vi "Set Properties from Initial.vi"(8 "error in(no error)":errorcluster, 10 "Initial Value":variant, 11 "Properties in":variant) -> (0 "error out":errorcluster, 2 "type":T1, 3 "Properties out":variant)   [LabVIEW 2020, in "Tag Engine Core.lvlib" / "Tag.lvclass"]
doc: "_SubVI_"
uses:
  Tag.lvclass
  <vilib>/Utility/Data Type/Type Definitions/Data Type.ctl
  Tag.lvclass/Tag.ctl
  <vilib>/Utility/Data Type/NI_Data Type.lvlib
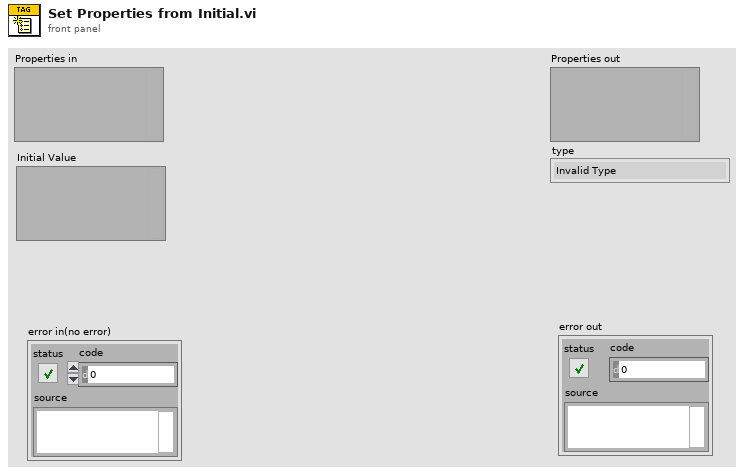
[diagram p1: front panel]
types:
  T1 = typedef "NI_Data Type.lvlib/Data Type.ctl" = enum8{"Invalid Type", "Void", "I8", "I16", "I32", "I64", "U8", "U16", "U32", "U64", "Single Float", "Double Float", "Extended Float", "Single Complex", "Double Complex", "Extended Complex", "Enum U8", "Enum U16", "Enum U32", "Enum U64", "Single Float With Unit", "Double Float With Unit", "Extended Float With Unit", "Single Complex with Unit", "Double Complex with Unit", "Extended Complex with Unit", "Boolean", "String", "Path", "Picture", "Tag", "Array", "Cluster", "Variant", "LV Variant", "Waveform", "Timestamp", "Digital Waveform", "Digital Data", "ExpressData", "Refnum", "External Data", "VI", "Poly VI", "LabVIEW Class Instance", "Fixed Point", "Set Collection", "Map Collection"}
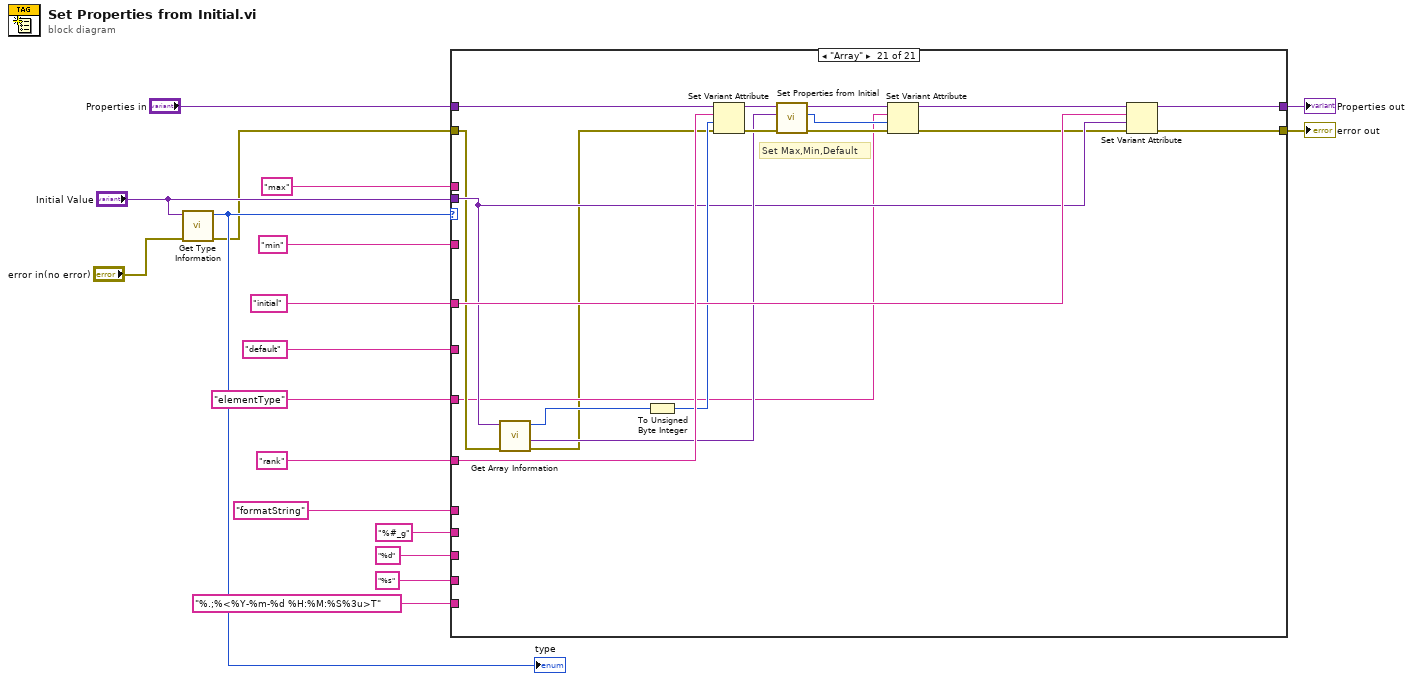
[diagram p0: block diagram]
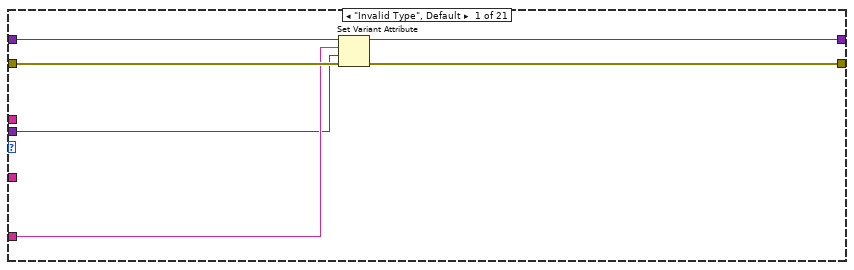
[diagram p2: hidden frame]
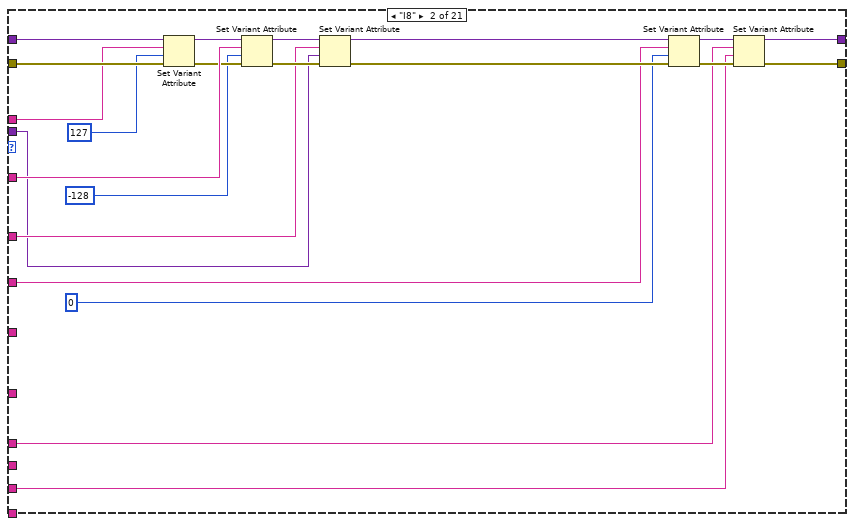
[diagram p3: hidden frame]
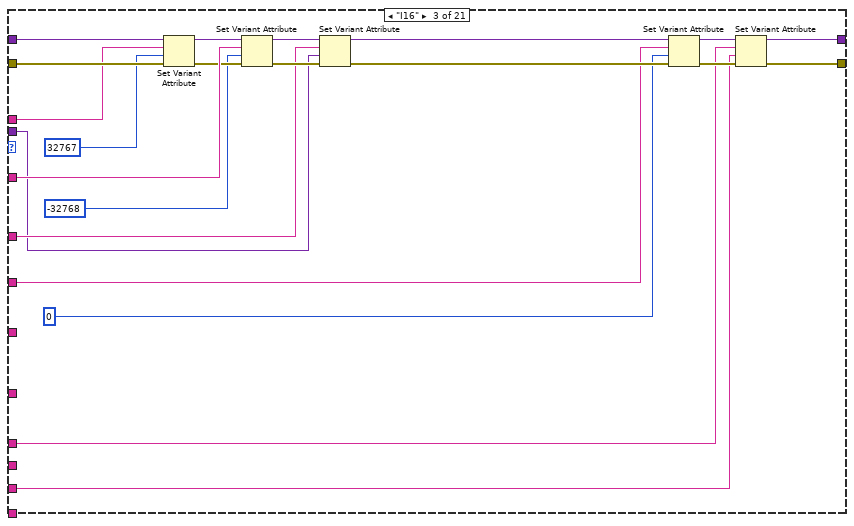
[diagram p4: hidden frame]
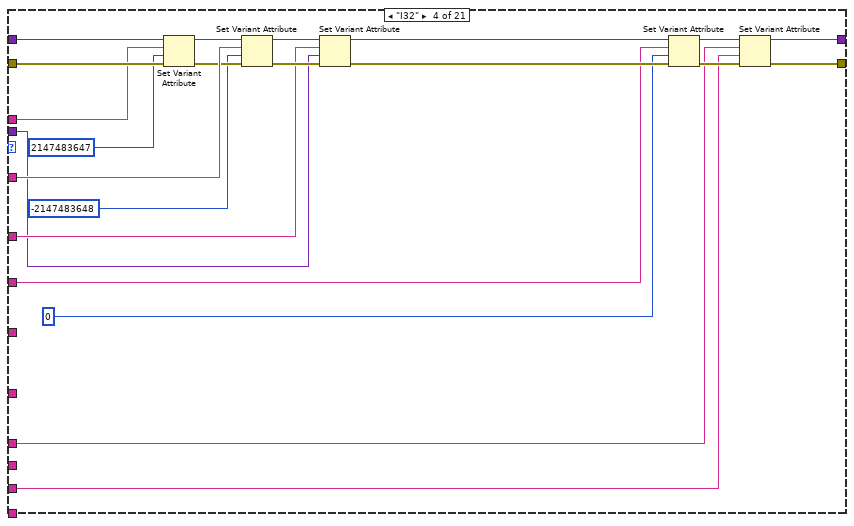
[diagram p5: hidden frame]
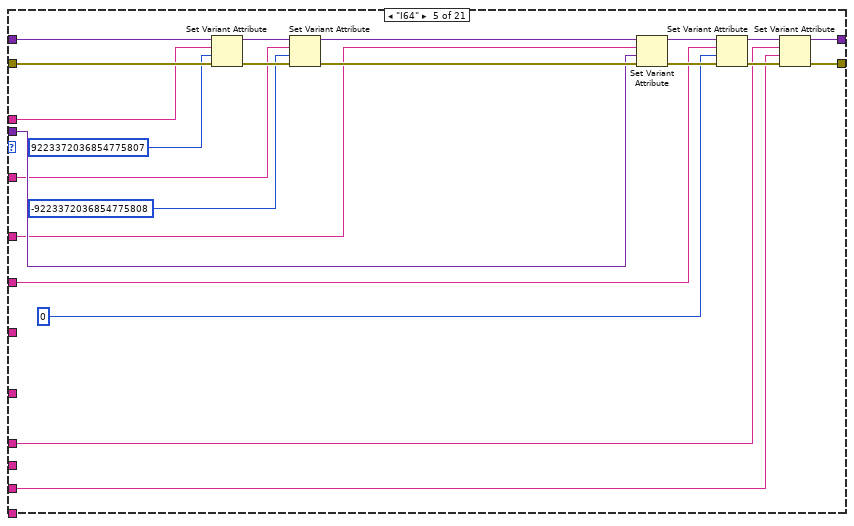
[diagram p6: hidden frame]
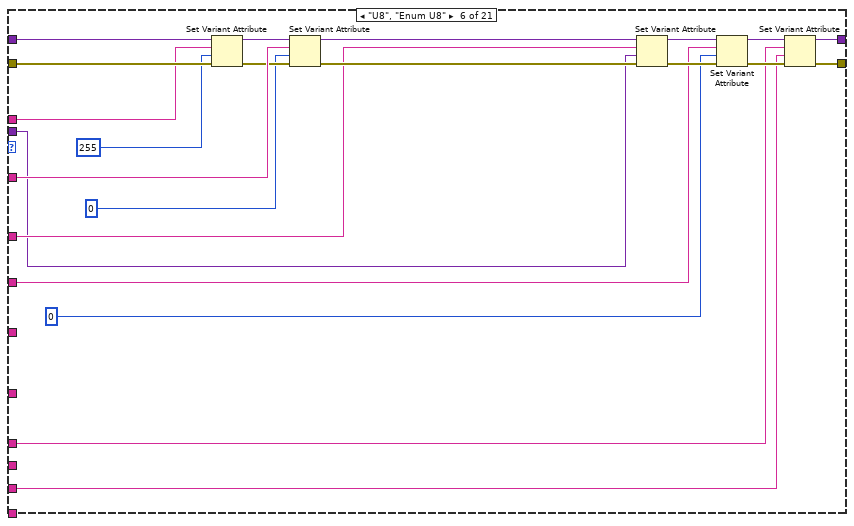
[diagram p7: hidden frame]
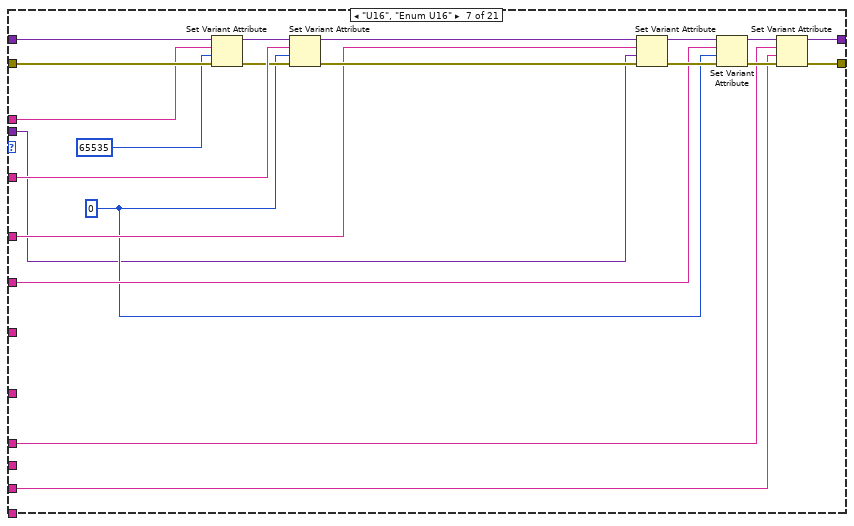
[diagram p8: hidden frame]
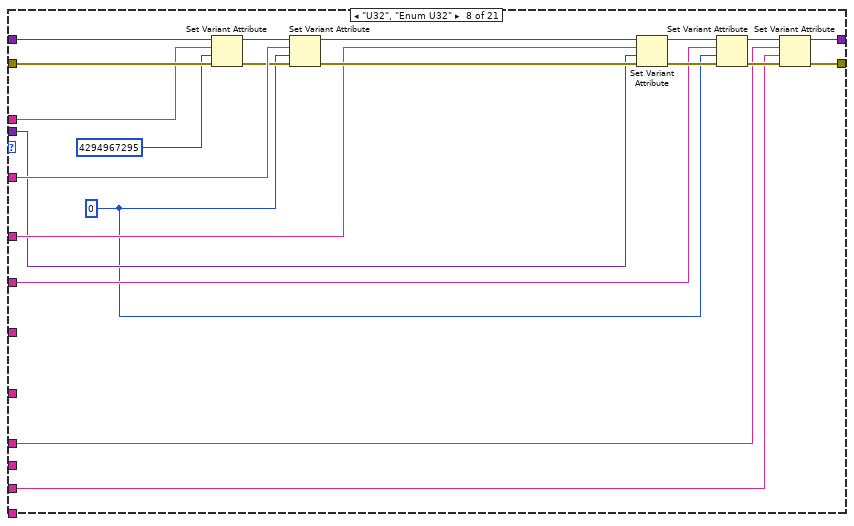
[diagram p9: hidden frame]
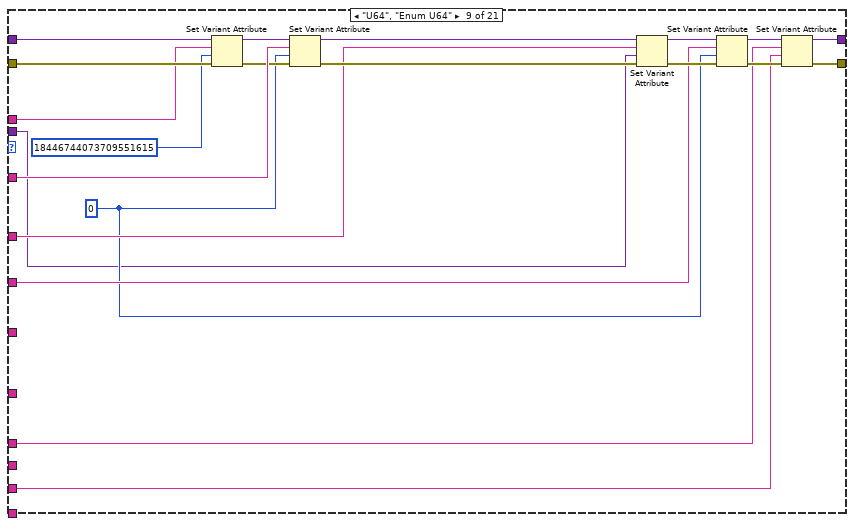
[diagram p10: hidden frame]
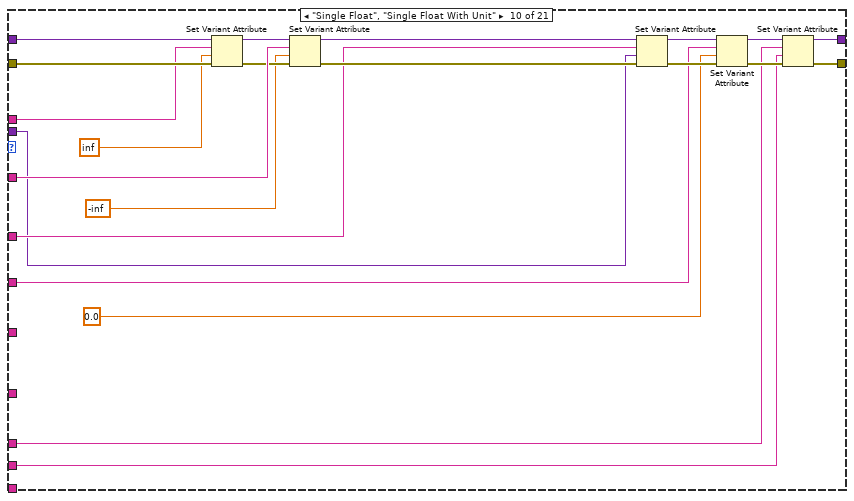
[diagram p11: hidden frame]
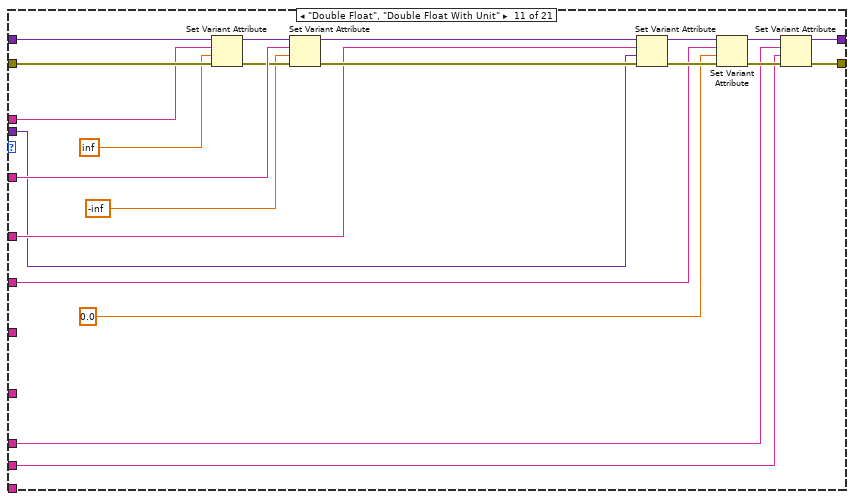
[diagram p12: hidden frame]
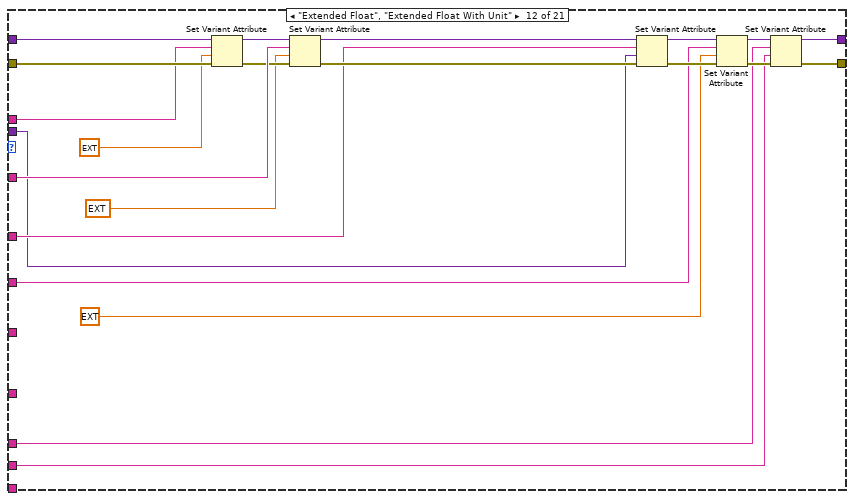
[diagram p13: hidden frame]
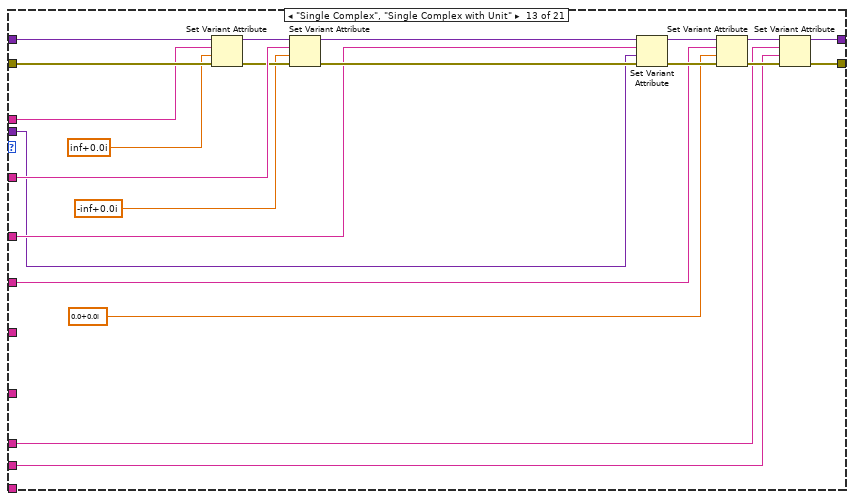
[diagram p14: hidden frame]
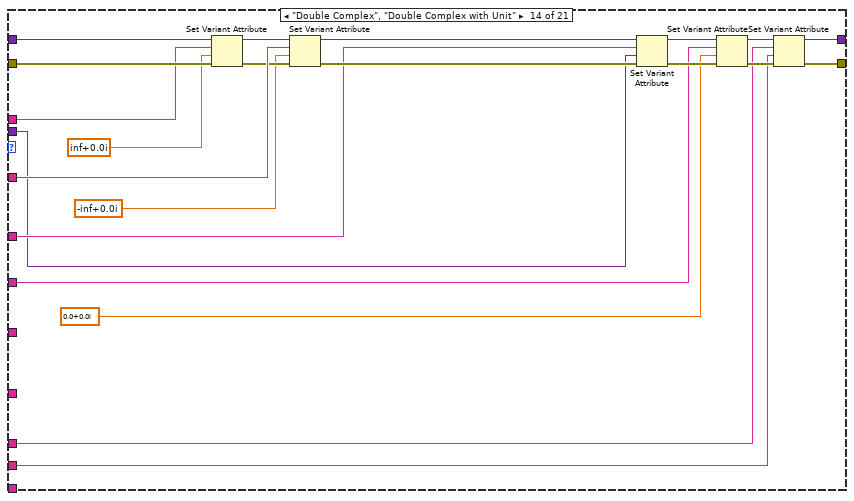
[diagram p15: hidden frame]
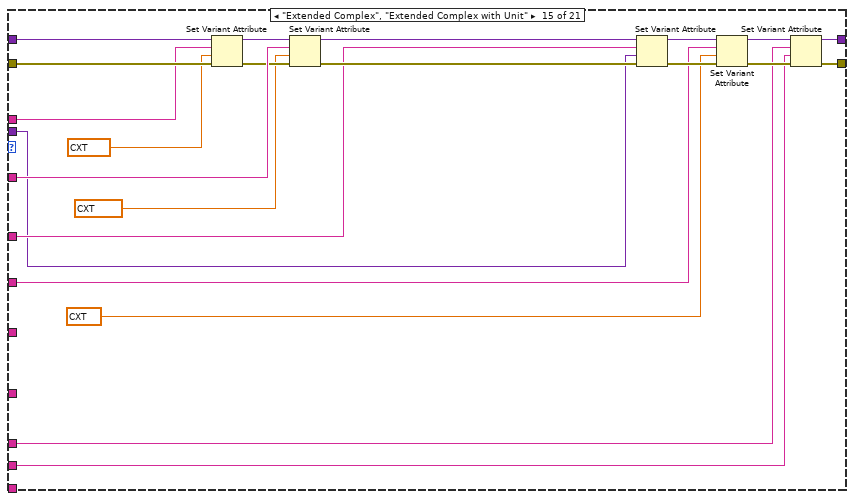
[diagram p16: hidden frame]
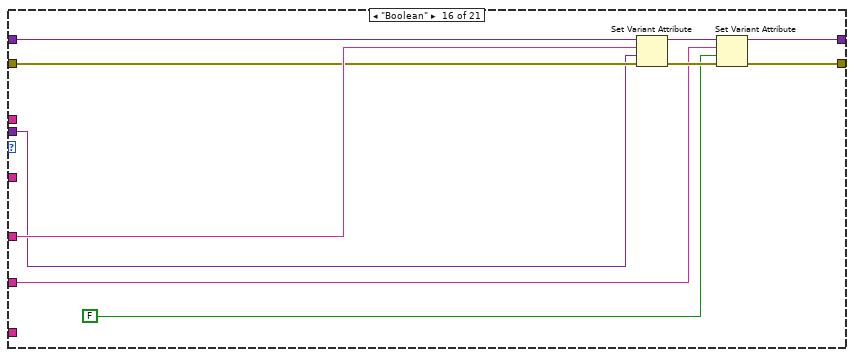
[diagram p17: hidden frame]
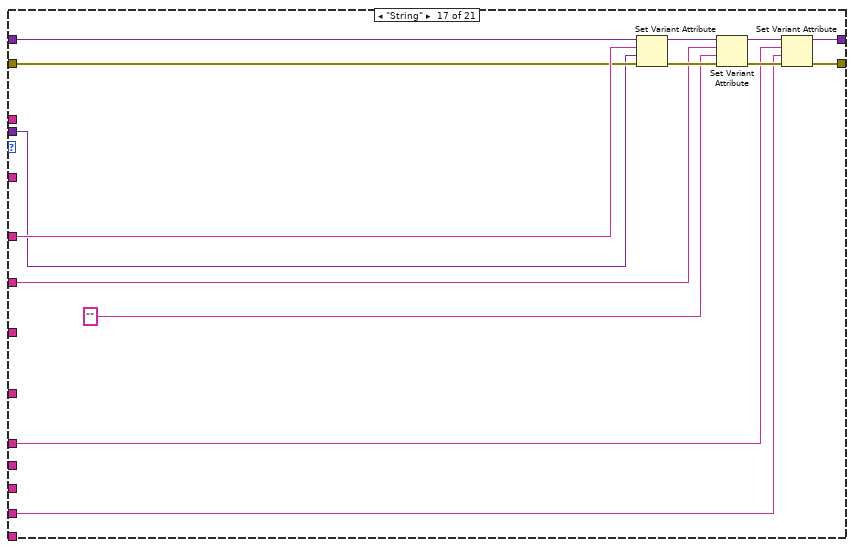
[diagram p18: hidden frame]
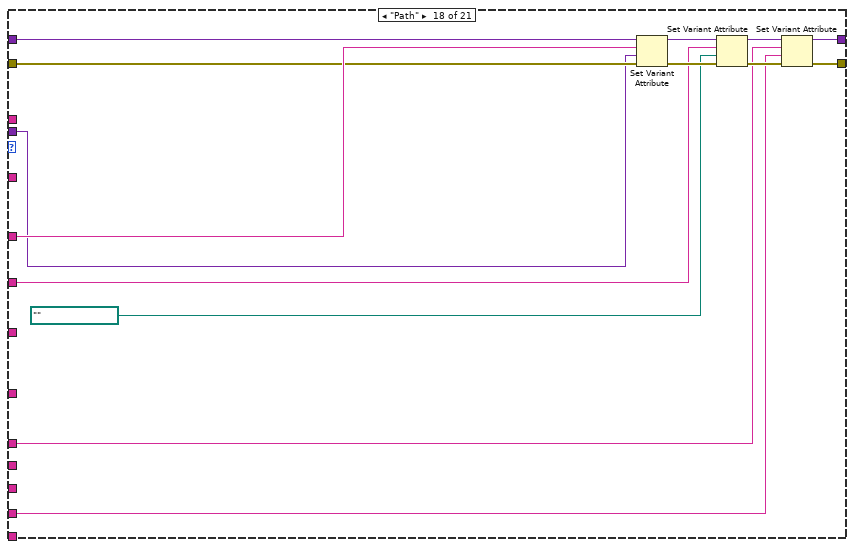
[diagram p19: hidden frame]
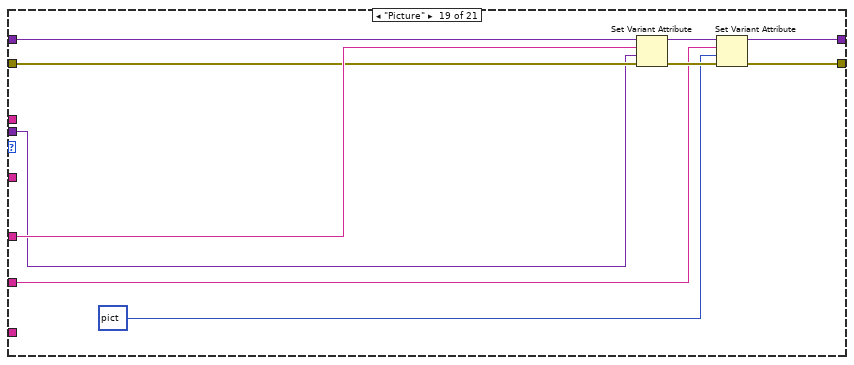
[diagram p20: hidden frame]
diagram:
  n1 = call <vilib>:"Get Type Information.vi"("error in (no error)"="error in(no error)", "variant"="Initial Value") -> ("error out"=w6:errorcluster, "type"=w8:T1)  [unwired: 5 in, 3 out]
  "type" <- w8
  n2 = case shown="\"Array\"" w8 {
    tunnel: "Properties in" -> [w24 w46 w68 w90 w112 w134 w155 w176 w197 w219 w241 w263 w285 w307 w329 w333 w349 w363 w371 w387 w400]
    tunnel: "Initial Value" -> [w19 w32 w53 w76 w103 w120 w141 w163 w183 w204 w226 w248 w271 w293 w314 w331 w347 w361 w369 w385 w401]
    tunnel: w6 -> [w23 w45 w67 w89 w111 w133 w154 w175 w196 w218 w240 w262 w284 w306 w328 w332 w348 w362 w370 w386 w399]
    tunnel: "max" ("$Path or Item Name") -> [_ w44 w66 w88 w101 w132 w153 w174 w195 w217 w239 w261 w283 w305 w327 _ _ _ _ _ _]
    tunnel: "min" ("$Path or Item Name") -> [_ w43 w65 w87 w100 w131 w152 w173 w194 w216 w238 w260 w282 w304 w326 _ _ _ _ _ _]
    tunnel: "initial" ("$Path or Item Name") -> [w22 w38 w60 w82 w99 w126 w147 w168 w189 w211 w233 w255 w277 w299 w321 w339 w353 w367 w377 w391 w407]
    tunnel: "default" ("$Path or Item Name") -> [_ w35 w57 w79 w98 w123 w144 w165 w186 w208 w230 w252 w274 w296 w318 w336 w350 w364 w374 w388 _]
    tunnel: [w21 w29 w48 w72 w94 w117 w136 w159 w180 w201 w223 w245 w267 w287 w311 w335 w343 w358 w373 w381 w406] -> w12
    tunnel: [w20 w27 w47 w71 w93 w115 w135 w158 w179 w200 w222 w244 w266 w286 w310 w334 w342 w357 w372 w380 w405] -> w11
    tunnel: "elementType" ("$Path or Item Name") -> [_ _ _ _ _ _ _ _ _ _ _ _ _ _ _ _ _ _ _ _ w395]
    tunnel: "rank" ("$Path or Item Name") -> [_ _ _ _ _ _ _ _ _ _ _ _ _ _ _ _ _ _ _ _ w410]
    tunnel: "formatString" -> [_ w26 w50 w70 w92 w114 w138 w157 w178 w199 w221 w243 w265 w289 w309 _ w341 w355 _ w378 _]
    tunnel: "%d" -> [_ w25 w49 w69 w91 w113 w137 w156 w177 _ _ _ _ _ _ _ _ _ _ _ _]
    tunnel: "%#_g" -> [_ _ _ _ _ _ _ _ _ w198 w220 w242 w264 w288 w308 _ _ _ _ _ _]
    tunnel: "%s" -> [_ _ _ _ _ _ _ _ _ _ _ _ _ _ _ _ w340 w354 _ _ _]
    tunnel: "%.;%<%Y-%m-%d %H:%M:%S%3u>T" -> [_ _ _ _ _ _ _ _ _ _ _ _ _ _ _ _ _ _ _ w379 _]
    frame "Invalid Type", Default {
      n3 = Set Variant Attribute(Variant=w24, name=w22, value=w19, error in=w23) -> (Variant out=w21:variant, error out=w20:errorcluster)  [unwired: 1 out]
    }
    frame "I8" {
      n4 = Set Variant Attribute(Variant=w46, name=w44, value=i8 127, error in=w45) -> (Variant out=w41:variant, error out=w42:errorcluster)  [unwired: 1 out]
      n5 = Set Variant Attribute(Variant=w41, name=w43, value=i8 -128, error in=w42) -> (Variant out=w39:variant, error out=w40:errorcluster)  [unwired: 1 out]
      n6 = Set Variant Attribute(Variant=w39, name=w38, value=w32, error in=w40) -> (Variant out=w37:variant, error out=w36:errorcluster)  [unwired: 1 out]
      n7 = Set Variant Attribute(Variant=w37, name=w35, value=i8 0, error in=w36) -> (Variant out=w30:variant, error out=w28:errorcluster)  [unwired: 1 out]
      n8 = Set Variant Attribute(Variant=w30, name=w26, value=w25, error in=w28) -> (Variant out=w29:variant, error out=w27:errorcluster)  [unwired: 1 out]
    }
    frame "I16" {
      n9 = Set Variant Attribute(Variant=w68, name=w66, value=i16 32767, error in=w67) -> (Variant out=w63:variant, error out=w64:errorcluster)  [unwired: 1 out]
      n10 = Set Variant Attribute(Variant=w63, name=w65, value=i16 -32768, error in=w64) -> (Variant out=w61:variant, error out=w62:errorcluster)  [unwired: 1 out]
      n11 = Set Variant Attribute(Variant=w61, name=w60, value=w53, error in=w62) -> (Variant out=w59:variant, error out=w58:errorcluster)  [unwired: 1 out]
      n12 = Set Variant Attribute(Variant=w59, name=w57, value=i16 0, error in=w58) -> (Variant out=w52:variant, error out=w51:errorcluster)  [unwired: 1 out]
      n13 = Set Variant Attribute(Variant=w52, name=w50, value=w49, error in=w51) -> (Variant out=w48:variant, error out=w47:errorcluster)  [unwired: 1 out]
    }
    frame "I32" {
      n14 = Set Variant Attribute(Variant=w90, name=w88, value=2147483647, error in=w89) -> (Variant out=w85:variant, error out=w86:errorcluster)  [unwired: 1 out]
      n15 = Set Variant Attribute(Variant=w85, name=w87, value=-2147483648, error in=w86) -> (Variant out=w83:variant, error out=w84:errorcluster)  [unwired: 1 out]
      n16 = Set Variant Attribute(Variant=w83, name=w82, value=w76, error in=w84) -> (Variant out=w81:variant, error out=w80:errorcluster)  [unwired: 1 out]
      n17 = Set Variant Attribute(Variant=w81, name=w79, value=0, error in=w80) -> (Variant out=w74:variant, error out=w73:errorcluster)  [unwired: 1 out]
      n18 = Set Variant Attribute(Variant=w74, name=w70, value=w69, error in=w73) -> (Variant out=w72:variant, error out=w71:errorcluster)  [unwired: 1 out]
    }
    frame "I64" {
      n19 = Set Variant Attribute(Variant=w112, name=w101, value=i64 9223372036854775807, error in=w111) -> (Variant out=w109:variant, error out=w110:errorcluster)  [unwired: 1 out]
      n20 = Set Variant Attribute(Variant=w109, name=w100, value=i64 -9223372036854775808, error in=w110) -> (Variant out=w97:variant, error out=w108:errorcluster)  [unwired: 1 out]
      n21 = Set Variant Attribute(Variant=w97, name=w99, value=w103, error in=w108) -> (Variant out=w107:variant, error out=w106:errorcluster)  [unwired: 1 out]
      n22 = Set Variant Attribute(Variant=w107, name=w98, value=i64 0, error in=w106) -> (Variant out=w96:variant, error out=w95:errorcluster)  [unwired: 1 out]
      n23 = Set Variant Attribute(Variant=w96, name=w92, value=w91, error in=w95) -> (Variant out=w94:variant, error out=w93:errorcluster)  [unwired: 1 out]
    }
    frame "U8", "Enum U8" {
      n24 = Set Variant Attribute(Variant=w134, name=w132, value=u8 255, error in=w133) -> (Variant out=w129:variant, error out=w130:errorcluster)  [unwired: 1 out]
      n25 = Set Variant Attribute(Variant=w129, name=w131, value=u8 0, error in=w130) -> (Variant out=w127:variant, error out=w128:errorcluster)  [unwired: 1 out]
      n26 = Set Variant Attribute(Variant=w127, name=w126, value=w120, error in=w128) -> (Variant out=w125:variant, error out=w124:errorcluster)  [unwired: 1 out]
      n27 = Set Variant Attribute(Variant=w125, name=w123, value=u8 0, error in=w124) -> (Variant out=w118:variant, error out=w116:errorcluster)  [unwired: 1 out]
      n28 = Set Variant Attribute(Variant=w118, name=w114, value=w113, error in=w116) -> (Variant out=w117:variant, error out=w115:errorcluster)  [unwired: 1 out]
    }
    frame "U16", "Enum U16" {
      w142 = u16 0
      n29 = Set Variant Attribute(Variant=w155, name=w153, value=u16 65535, error in=w154) -> (Variant out=w150:variant, error out=w151:errorcluster)  [unwired: 1 out]
      n30 = Set Variant Attribute(Variant=w150, name=w152, value=w142, error in=w151) -> (Variant out=w148:variant, error out=w149:errorcluster)  [unwired: 1 out]
      n31 = Set Variant Attribute(Variant=w148, name=w147, value=w141, error in=w149) -> (Variant out=w146:variant, error out=w145:errorcluster)  [unwired: 1 out]
      n32 = Set Variant Attribute(Variant=w146, name=w144, value=w142, error in=w145) -> (Variant out=w140:variant, error out=w139:errorcluster)  [unwired: 1 out]
      n33 = Set Variant Attribute(Variant=w140, name=w138, value=w137, error in=w139) -> (Variant out=w136:variant, error out=w135:errorcluster)  [unwired: 1 out]
    }
    frame "U32", "Enum U32" {
      w162 = u32 0
      n34 = Set Variant Attribute(Variant=w176, name=w174, value=u32 4294967295, error in=w175) -> (Variant out=w171:variant, error out=w172:errorcluster)  [unwired: 1 out]
      n35 = Set Variant Attribute(Variant=w171, name=w173, value=w162, error in=w172) -> (Variant out=w169:variant, error out=w170:errorcluster)  [unwired: 1 out]
      n36 = Set Variant Attribute(Variant=w169, name=w168, value=w163, error in=w170) -> (Variant out=w167:variant, error out=w166:errorcluster)  [unwired: 1 out]
      n37 = Set Variant Attribute(Variant=w167, name=w165, value=w162, error in=w166) -> (Variant out=w161:variant, error out=w160:errorcluster)  [unwired: 1 out]
      n38 = Set Variant Attribute(Variant=w161, name=w157, value=w156, error in=w160) -> (Variant out=w159:variant, error out=w158:errorcluster)  [unwired: 1 out]
    }
    frame "U64", "Enum U64" {
      w184 = u64 0
      n39 = Set Variant Attribute(Variant=w197, name=w195, value=u64 18446744073709551615, error in=w196) -> (Variant out=w192:variant, error out=w193:errorcluster)  [unwired: 1 out]
      n40 = Set Variant Attribute(Variant=w192, name=w194, value=w184, error in=w193) -> (Variant out=w190:variant, error out=w191:errorcluster)  [unwired: 1 out]
      n41 = Set Variant Attribute(Variant=w190, name=w189, value=w183, error in=w191) -> (Variant out=w188:variant, error out=w187:errorcluster)  [unwired: 1 out]
      n42 = Set Variant Attribute(Variant=w188, name=w186, value=w184, error in=w187) -> (Variant out=w182:variant, error out=w181:errorcluster)  [unwired: 1 out]
      n43 = Set Variant Attribute(Variant=w182, name=w178, value=w177, error in=w181) -> (Variant out=w180:variant, error out=w179:errorcluster)  [unwired: 1 out]
    }
    frame "Single Float", "Single Float With Unit" {
      n44 = Set Variant Attribute(Variant=w219, name=w217, value=sgl inf, error in=w218) -> (Variant out=w214:variant, error out=w215:errorcluster)  [unwired: 1 out]
      n45 = Set Variant Attribute(Variant=w214, name=w216, value=sgl -inf, error in=w215) -> (Variant out=w212:variant, error out=w213:errorcluster)  [unwired: 1 out]
      n46 = Set Variant Attribute(Variant=w212, name=w211, value=w204, error in=w213) -> (Variant out=w210:variant, error out=w209:errorcluster)  [unwired: 1 out]
      n47 = Set Variant Attribute(Variant=w210, name=w208, value=sgl 0.0, error in=w209) -> (Variant out=w203:variant, error out=w202:errorcluster)  [unwired: 1 out]
      n48 = Set Variant Attribute(Variant=w203, name=w199, value=w198, error in=w202) -> (Variant out=w201:variant, error out=w200:errorcluster)  [unwired: 1 out]
    }
    frame "Double Float", "Double Float With Unit" {
      n49 = Set Variant Attribute(Variant=w241, name=w239, value=inf, error in=w240) -> (Variant out=w236:variant, error out=w237:errorcluster)  [unwired: 1 out]
      n50 = Set Variant Attribute(Variant=w236, name=w238, value=-inf, error in=w237) -> (Variant out=w234:variant, error out=w235:errorcluster)  [unwired: 1 out]
      n51 = Set Variant Attribute(Variant=w234, name=w233, value=w226, error in=w235) -> (Variant out=w232:variant, error out=w231:errorcluster)  [unwired: 1 out]
      n52 = Set Variant Attribute(Variant=w232, name=w230, value=0.0, error in=w231) -> (Variant out=w225:variant, error out=w224:errorcluster)  [unwired: 1 out]
      n53 = Set Variant Attribute(Variant=w225, name=w221, value=w220, error in=w224) -> (Variant out=w223:variant, error out=w222:errorcluster)  [unwired: 1 out]
    }
    frame "Extended Float", "Extended Float With Unit" {
      n54 = Set Variant Attribute(Variant=w263, name=w261, value=ext inf, error in=w262) -> (Variant out=w258:variant, error out=w259:errorcluster)  [unwired: 1 out]
      n55 = Set Variant Attribute(Variant=w258, name=w260, value=ext -inf, error in=w259) -> (Variant out=w256:variant, error out=w257:errorcluster)  [unwired: 1 out]
      n56 = Set Variant Attribute(Variant=w256, name=w255, value=w248, error in=w257) -> (Variant out=w254:variant, error out=w253:errorcluster)  [unwired: 1 out]
      n57 = Set Variant Attribute(Variant=w254, name=w252, value=ext 0.0, error in=w253) -> (Variant out=w247:variant, error out=w246:errorcluster)  [unwired: 1 out]
      n58 = Set Variant Attribute(Variant=w247, name=w243, value=w242, error in=w246) -> (Variant out=w245:variant, error out=w244:errorcluster)  [unwired: 1 out]
    }
    frame "Single Complex", "Single Complex with Unit" {
      n59 = Set Variant Attribute(Variant=w285, name=w283, value=csg inf+0.0i, error in=w284) -> (Variant out=w280:variant, error out=w281:errorcluster)  [unwired: 1 out]
      n60 = Set Variant Attribute(Variant=w280, name=w282, value=csg -inf+0.0i, error in=w281) -> (Variant out=w278:variant, error out=w279:errorcluster)  [unwired: 1 out]
      n61 = Set Variant Attribute(Variant=w278, name=w277, value=w271, error in=w279) -> (Variant out=w276:variant, error out=w275:errorcluster)  [unwired: 1 out]
      n62 = Set Variant Attribute(Variant=w276, name=w274, value=csg 0.0+0.0i, error in=w275) -> (Variant out=w269:variant, error out=w268:errorcluster)  [unwired: 1 out]
      n63 = Set Variant Attribute(Variant=w269, name=w265, value=w264, error in=w268) -> (Variant out=w267:variant, error out=w266:errorcluster)  [unwired: 1 out]
    }
    frame "Double Complex", "Double Complex with Unit" {
      n64 = Set Variant Attribute(Variant=w307, name=w305, value=cdb inf+0.0i, error in=w306) -> (Variant out=w302:variant, error out=w303:errorcluster)  [unwired: 1 out]
      n65 = Set Variant Attribute(Variant=w302, name=w304, value=cdb -inf+0.0i, error in=w303) -> (Variant out=w300:variant, error out=w301:errorcluster)  [unwired: 1 out]
      n66 = Set Variant Attribute(Variant=w300, name=w299, value=w293, error in=w301) -> (Variant out=w298:variant, error out=w297:errorcluster)  [unwired: 1 out]
      n67 = Set Variant Attribute(Variant=w298, name=w296, value=cdb 0.0+0.0i, error in=w297) -> (Variant out=w291:variant, error out=w290:errorcluster)  [unwired: 1 out]
      n68 = Set Variant Attribute(Variant=w291, name=w289, value=w288, error in=w290) -> (Variant out=w287:variant, error out=w286:errorcluster)  [unwired: 1 out]
    }
    frame "Extended Complex", "Extended Complex with Unit" {
      n69 = Set Variant Attribute(Variant=w329, name=w327, value=cxt inf+0.0i, error in=w328) -> (Variant out=w324:variant, error out=w325:errorcluster)  [unwired: 1 out]
      n70 = Set Variant Attribute(Variant=w324, name=w326, value=cxt -inf+0.0i, error in=w325) -> (Variant out=w322:variant, error out=w323:errorcluster)  [unwired: 1 out]
      n71 = Set Variant Attribute(Variant=w322, name=w321, value=w314, error in=w323) -> (Variant out=w320:variant, error out=w319:errorcluster)  [unwired: 1 out]
      n72 = Set Variant Attribute(Variant=w320, name=w318, value=cxt 0.0+0.0i, error in=w319) -> (Variant out=w313:variant, error out=w312:errorcluster)  [unwired: 1 out]
      n73 = Set Variant Attribute(Variant=w313, name=w309, value=w308, error in=w312) -> (Variant out=w311:variant, error out=w310:errorcluster)  [unwired: 1 out]
    }
    frame "Boolean" {
      n74 = Set Variant Attribute(Variant=w333, name=w339, value=w331, error in=w332) -> (Variant out=w338:variant, error out=w337:errorcluster)  [unwired: 1 out]
      n75 = Set Variant Attribute(Variant=w338, name=w336, value=FALSE, error in=w337) -> (Variant out=w335:variant, error out=w334:errorcluster)  [unwired: 1 out]
    }
    frame "String" {
      n76 = Set Variant Attribute(Variant=w349, name=w353, value=w347, error in=w348) -> (Variant out=w352:variant, error out=w351:errorcluster)  [unwired: 1 out]
      n77 = Set Variant Attribute(Variant=w352, name=w350, value="", error in=w351) -> (Variant out=w345:variant, error out=w344:errorcluster)  [unwired: 1 out]
      n78 = Set Variant Attribute(Variant=w345, name=w341, value=w340, error in=w344) -> (Variant out=w343:variant, error out=w342:errorcluster)  [unwired: 1 out]
    }
    frame "Path" {
      n79 = Set Variant Attribute(Variant=w363, name=w367, value=w361, error in=w362) -> (Variant out=w366:variant, error out=w365:errorcluster)  [unwired: 1 out]
      n80 = Set Variant Attribute(Variant=w366, name=w364, value=path "", error in=w365) -> (Variant out=w359:variant, error out=w356:errorcluster)  [unwired: 1 out]
      n81 = Set Variant Attribute(Variant=w359, name=w355, value=w354, error in=w356) -> (Variant out=w358:variant, error out=w357:errorcluster)  [unwired: 1 out]
    }
    frame "Picture" {
      n82 = Set Variant Attribute(Variant=w371, name=w377, value=w369, error in=w370) -> (Variant out=w376:variant, error out=w375:errorcluster)  [unwired: 1 out]
      n83 = Set Variant Attribute(Variant=w376, name=w374, value=picture data[5B] ("empty picture"), error in=w375) -> (Variant out=w373:variant, error out=w372:errorcluster)  [unwired: 1 out]
    }
    frame "Timestamp" {
      n84 = Set Variant Attribute(Variant=w387, name=w391, value=w385, error in=w386) -> (Variant out=w390:variant, error out=w389:errorcluster)  [unwired: 1 out]
      n85 = Set Variant Attribute(Variant=w390, name=w388, value=timestamp(0 s since 1904-01-01), error in=w389) -> (Variant out=w383:variant, error out=w382:errorcluster)  [unwired: 1 out]
      n86 = Set Variant Attribute(Variant=w383, name=w378, value=w379, error in=w382) -> (Variant out=w381:variant, error out=w380:errorcluster)  [unwired: 1 out]
    }
    frame "Array" {
      # "Set Max,Min,Default"
      n87 = call <vilib>:"Get Array Information.vi"("error in (no error)"=w399, "variant"=w401) -> ("error out"=w394:errorcluster, "array element data type"=w402:variant, "number of dimensions"=w404:i32)  [unwired: 6 in, 1 out]
      n88 = To Unsigned Byte Integer(number=w404) -> (unsigned 8bit integer=w403:u8)
      n89 = Set Variant Attribute(Variant=w400, name=w410, value=w403, error in=w394) -> (Variant out=w409:variant, error out=w408:errorcluster)  [unwired: 1 out]
      n90 = call "Set Properties from Initial.vi"("error in(no error)"=w408, "Initial Value"=w402, "Properties in"=w409) -> ("error out"=w397:errorcluster, "type"=w396:T1, "Properties out"=w398:variant)  [unwired: 6 in]
      n91 = Set Variant Attribute(Variant=w398, name=w395, value=w396, error in=w397) -> (Variant out=w392:variant, error out=w393:errorcluster)  [unwired: 1 out]
      n92 = Set Variant Attribute(Variant=w392, name=w407, value=w401, error in=w393) -> (Variant out=w406:variant, error out=w405:errorcluster)  [unwired: 1 out]
    }
  }
  "Properties out" <- w12
  "error out" <- w11
